vi "Build Toast With Classes.vi"(8 "error in":errorcluster) -> (0 "error out":errorcluster, 3 "Toast XML":string)   [LabVIEW 2026]
doc: "Development example for displaying a notification from a ToastBuilder or an XML string through ToastService. The base ActivationHandler performs no application action. Press Stop to close the service and source."
uses:
  ActivationHandler/ActivationHandler.lvclass
  ToastBuilder/ToastBuilder.lvclass
  ToastBuilder/Create ToastBuilder.vi
  ToastFromXML/Create ToastFromXML.vi
  ToastSource/ToastSource.lvclass
  ToastFromXML/ToastFromXML.lvclass
  ToastService/ToastService.lvclass
  ToastNotification/ToastNotification.lvlib
panel:
  in  "stop":bool
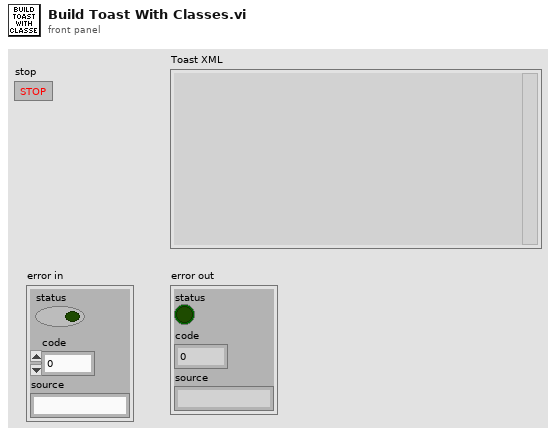
[diagram p1: front panel]
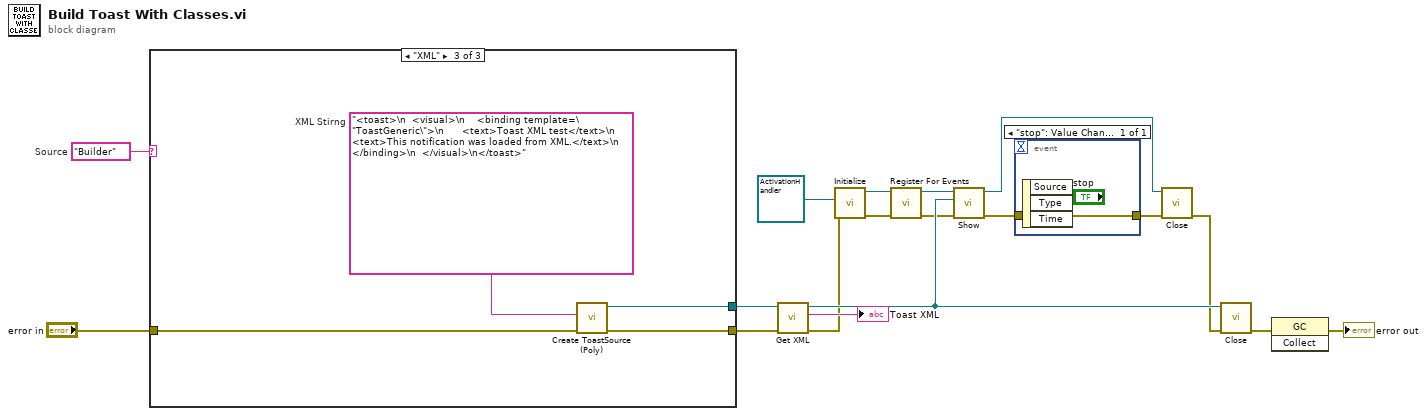
[diagram p0: block diagram]
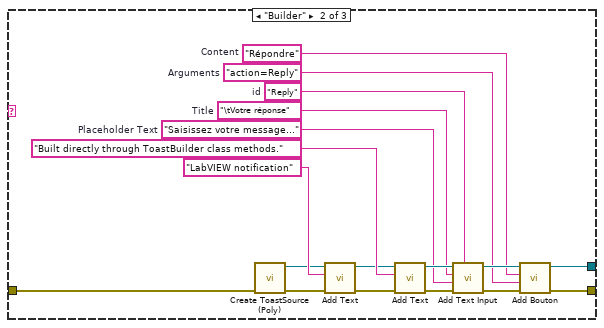
[diagram p3: hidden frame]
diagram:
  w1 = "Builder"  # Source
  n1 = case shown="\"XML\"" w1 {
    tunnel: "error in" -> [w19 w31 w41]
    tunnel: [w19 w24 w40] -> w4
    tunnel: [_ w22 w39] -> w3
    frame Default {
    }
    frame "Builder" {
      w20 = "action=Reply"  # Arguments
      w21 = "Répondre"  # Content
      w26 = "Saisissez votre message…"  # Placeholder Text
      w27 = "\tVotre réponse"  # Title
      w28 = "Reply"  # id
      n2 = call-poly "Create ToastSource (Poly).vi"("error in"=w31) -> ("error out"=w33:errorcluster, "ToastBuilder out"=w32:refnum<class "ToastBuilder.lvclass">)  [unwired: 9 in]
      n3 = call "Add Text.vi"("error in"=w33, "text"="LabVIEW notification", "ToastBuilder in"=w32) -> ("error out"=w36:errorcluster, "ToastBuilder out"=w35:refnum<class "ToastBuilder.lvclass">)  [unwired: 7 in]
      n4 = call "Add Text.vi"("error in"=w36, "text"="Built directly through ToastBuilder class methods.", "ToastBuilder in"=w35) -> ("error out"=w29:errorcluster, "ToastBuilder out"=w30:refnum<class "ToastBuilder.lvclass">)  [unwired: 7 in]
      n5 = call "Add Text Input.vi"("id"=w28, "error in (no error)"=w29, "Placeholder Text"=w26, "Title"=w27, "ToastBuilder in"=w30) -> ("error out"=w25:errorcluster, "ToastBuilder out"=w23:refnum<class "ToastBuilder.lvclass">)  [unwired: 5 in]
      n6 = call "Add Bouton.vi"("error in (no error)"=w25, "Arguments"=w20, "Content"=w21, "ToastBuilder in"=w23) -> ("error out"=w24:errorcluster, "ToastBuilder out"=w22:refnum<class "ToastBuilder.lvclass">)  [unwired: 6 in]
    }
    frame "XML" {
      w38 = "<toast>\n  <visual>\n    <binding template=\"ToastGeneric\">\n      <text>Toast XML test</text>\n      <text>This notification was loaded from XML.</text>\n    </binding>\n  </visual>\n</toast>"  # XML Stirng
      n7 = call-poly "Create ToastSource (Poly).vi"("error in (no error)"=w41, "XML Stirng"=w38) -> ("error out"=w40:errorcluster, "ToastFromXML out"=w39:refnum<class "ToastFromXML.lvclass">)  [unwired: 8 in]
    }
  }
  n8 = call-dynamic "Get XML.vi"("error in (no error)"=w4, "ToastSource in"=w3) -> ("error out"=w15:errorcluster, "GetContent"=→"Toast XML":string, "ToastSource out"=w16:refnum<class "ToastSource.lvclass">)  [unwired: 7 in]
  n9 = call "Initialize.vi"("error in (no error)"=w15, "ActivationHandler in"=refnum<class "ActivationHandler.lvclass"> refnum) -> ("error out"=w13:errorcluster, "ToastService out"=w11:refnum<class "ToastService.lvclass">)  [unwired: 7 in, 1 out]
  n10 = call "Register For Events.vi"("error in (no error)"=w13, "ToastService in"=w11) -> ("error out"=w12:errorcluster, "ToastService out"=w10:refnum<class "ToastService.lvclass">)  [unwired: 8 in]
  n11 = call "Show.vi"("error in (no error)"=w12, "ToastSource in"=w16, "ToastService in"=w10) -> ("error out"=w9:errorcluster, "ToastService out"=w7:refnum<class "ToastService.lvclass">)  [unwired: 7 in]
  n12 = event shown="[0] \"stop\": Value Change" {
    selector: _ -> [_]
    dyn-events: _ -> [_]
    timeout: _ -> [_]
    tunnel: [w42] -> w8
    tunnel: w9 -> [w42]
    event "stop": Value Change {
      n13 = event-data() -> ()  [unwired: 1 in, 3 out]
    }
  }
  n14 = call "Close.vi"("error in (no error)"=w8, "ToastService in"=w7) -> ("error out"=w14:errorcluster)  [unwired: 9 in]
  n15 = call-dynamic "Close.vi"("error in (no error)"=w14, "ToastSource in"=w16) -> ("error out"=w6:errorcluster)  [unwired: 9 in]
  n16 = invoke class="GC" method="Collect"(error in=w6) -> (error out=→"error out":errorcluster)  [unwired: 2 in, 2 out]
